vi "Find Account.vi"(8 "error in":errorcluster, 10 "Account Number":string, 11 "Accounts":T1[](array[typedef])) -> (0 "error out":errorcluster, 1 "Index":i32, 2 "Account":T1, 3 "Account Found?":bool)   [LabVIEW 2026]
doc: "Searches an array of ATM Account records for the given Account Number. Both the searched number and the stored numbers are trimmed of whitespace and compared exactly. Returns Account Found? TRUE with the record and its array index, or FALSE with an empty record and Index -1. Pure function, no file access; error in is passed through to error out."
uses:
  <vilib>/Utility/error.llb/Trim Whitespace (string).vi
  <vilib>/Utility/error.llb/Trim Whitespace One-Sided.vi
  Controls/ATM Account.ctl
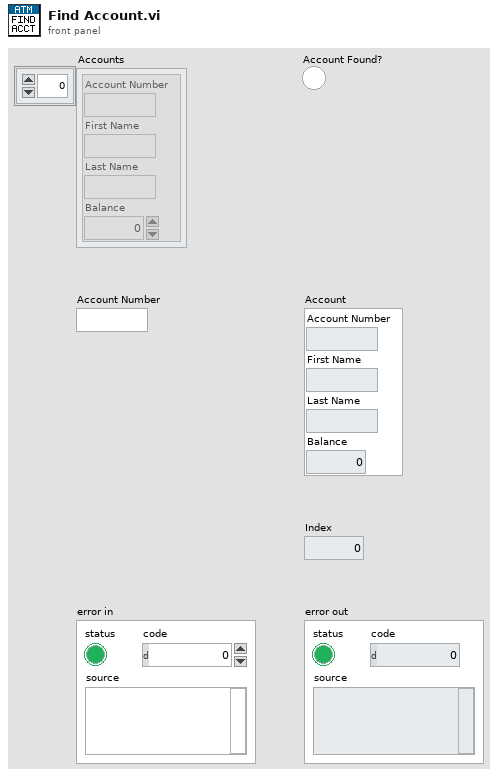
[diagram p1: front panel]
types:
  T1 = typedef "ATM Account.ctl" = cluster{"Account Number":string, "First Name":string, "Last Name":string, "Balance":dbl}
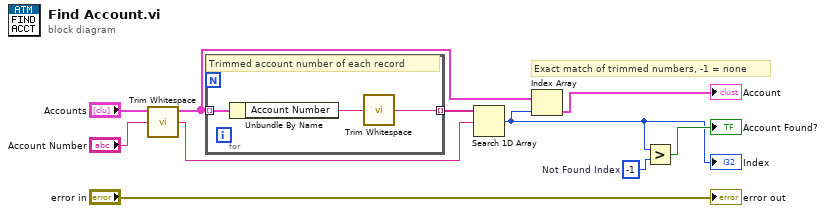
[diagram p0: block diagram]
diagram:
  w6 = -1  # Not Found Index
  # "Exact match of trimmed numbers, -1 = none"
  n1 = call-poly <vilib>:"Trim Whitespace.vi"("string"="Account Number") -> ("trimmed string"=w7:string)  [unwired: 1 in]
  n2 = for {
    tunnel: "Accounts" -> [w12] mode=indexing
    tunnel: [w10] -> w8 mode=indexing
    # "Trimmed account number of each record"
    n3 = Unbundle By Name(w12) -> ("Account Number"=w11:string)
    n4 = call-poly <vilib>:"Trim Whitespace.vi"("string"=w11) -> ("trimmed string"=w10:string)  [unwired: 1 in]
  }
  n5 = Search 1D Array(1D array=w8, element=w7) -> (index of element=w2:i32)  [unwired: 1 in]
  "Index" <- w2
  n6 = Index Array(array="Accounts", index=w2) -> (element=→"Account":T1)
  n7 = Greater?(x=w2, y=w6) -> (0:→"Account Found?":bool)
  "error out" <- "error in"
